vi "MalformedMessageReceivedEvent.vi"(4 "FromListener":refnum<vi>, 5 "事件数据":cluster{"source":refnum<k24>, "message":string}, 6 "控件引用":refnum<k24>, 7 "事件通用数据":cluster{"事件源":i32, "事件类型":u32, "时间标识":u32}) -> ()   [LabVIEW 2018]
uses:
  C:/users data/project/MES/MES v4.5 20250917/module/CFX/CFX_dll/CFX.dll
  CFX_dll/CFX.dll
panel:
  out "错误输出":errorcluster
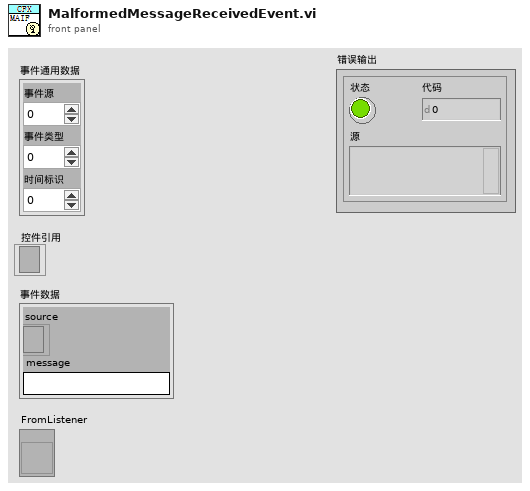
[diagram p1: front panel]
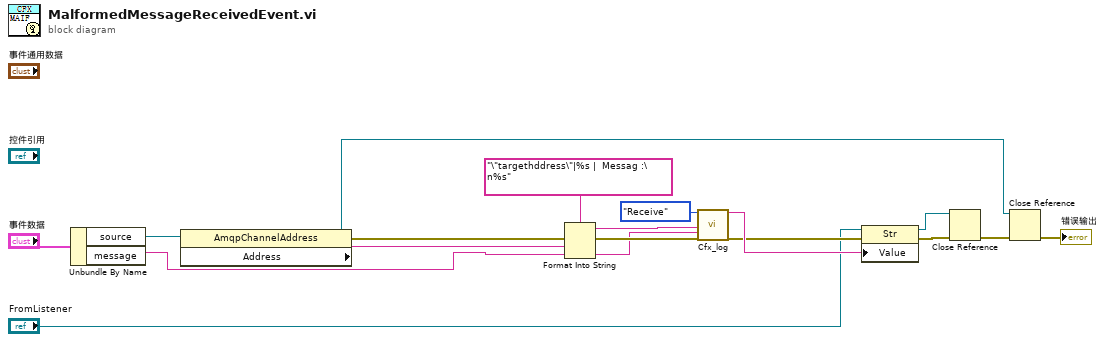
[diagram p0: block diagram]
diagram:
  n1 = Unbundle By Name("事件数据") -> ("source"=w5:refnum<k24>, "message"=w4:string)
  n2 = property on="属性节点" class="AmqpChannelAddress"(reference=w5) -> (reference out=w3:refnum<k24>, error out=w2:errorcluster, "Address"=w9:string)  [unwired: 1 in]
  n3 = Format Into String(format string="\"targethddress\"|%s |  Messag :\n%s" ("格式字符串"), error in=w2, w9, w4) -> (resulting string=w10:string, error out=w7:errorcluster)  [unwired: 1 in]
  n4 = call "Cfx_log.vi"("R/W"=enum16{"Send", "Receive"}."Receive", "Message_Name"=w10, "Message_Content"=w4, "error in"=w7) -> ("Log_out"=w12:string, "error out"=w11:errorcluster)  [unwired: 14 in]
  n5 = property on="属性节点" class="Str"(reference="FromListener", error in=w11, "Value"=w12) -> (reference out=w16:refnum<vi>, error out=w15:errorcluster)
  n6 = Close Reference(reference=w16, error in (no error)=w15) -> (error out=w14:errorcluster)
  n7 = Close Reference(reference=w3, error in (no error)=w14) -> (error out=→"错误输出":errorcluster)
